vi "Signal CP Assigned Table.vi"(8 "CP Probability":dbl[][](array[numeric]), 9 "time":dbl[](array[numeric]), 10 "Change Point Array":T2, 11 "Assigned CP Profile plus":T1) -> (3 "CP Profile Table":string[][](table) caption="CP Table")   [LabVIEW 2018]
panel:
  out "サイズ 3":i32
  out "配列":string[][](array[string])
  out "要素":i32
  out "サイズ 2":i32
  out "サイズ":i32[](array[numeric])
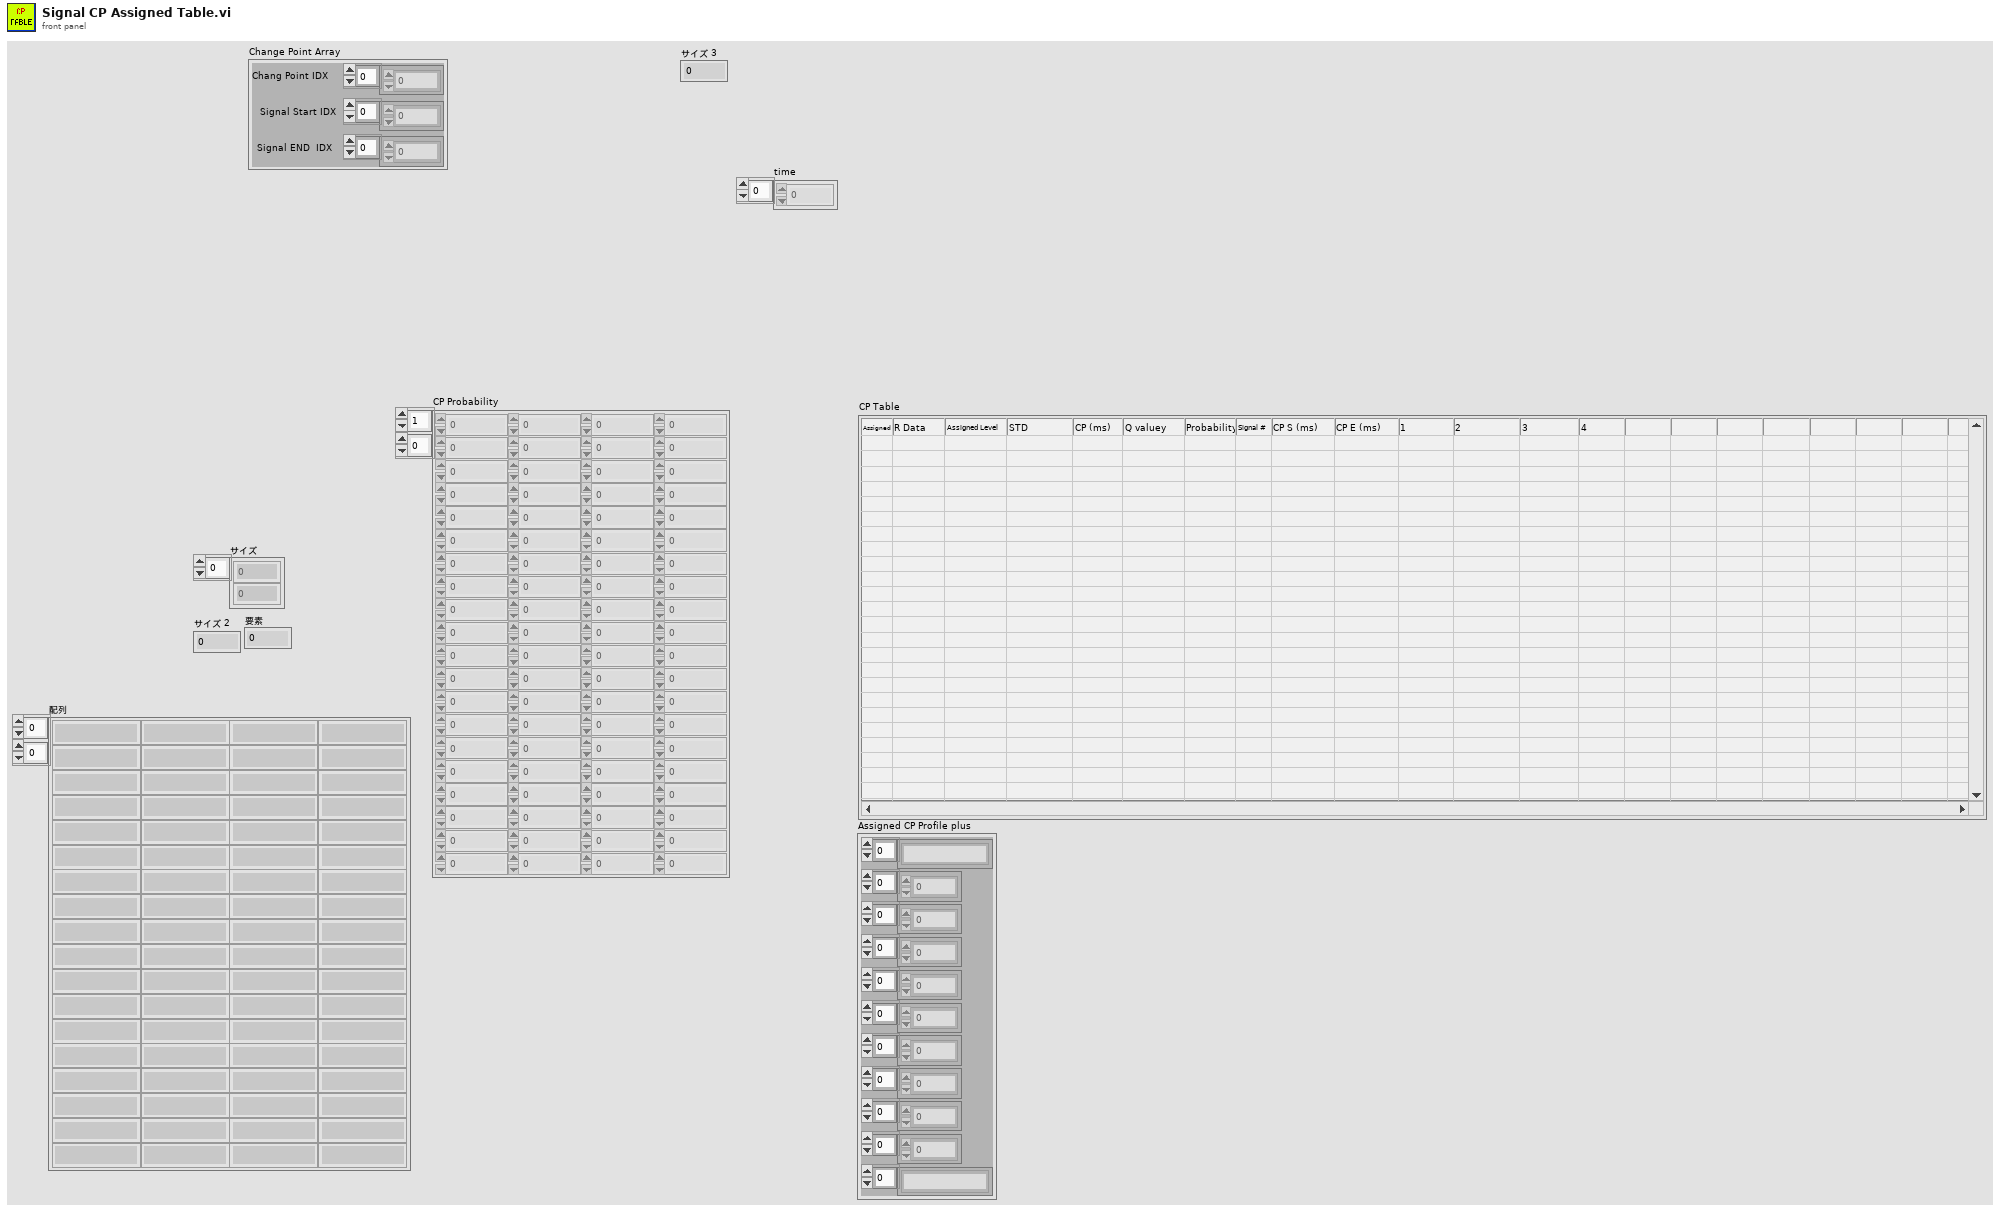
[diagram p1: front panel]
types:
  T1 = cluster{string[], dbl[], dbl[], dbl[], i32[], dbl[], dbl[], i32[], i32[], i32[], string[]}
  T2 = cluster{"Chang Point IDX":i32[], "Signal Start IDX":i32[], "Signal END  IDX":i32[]}
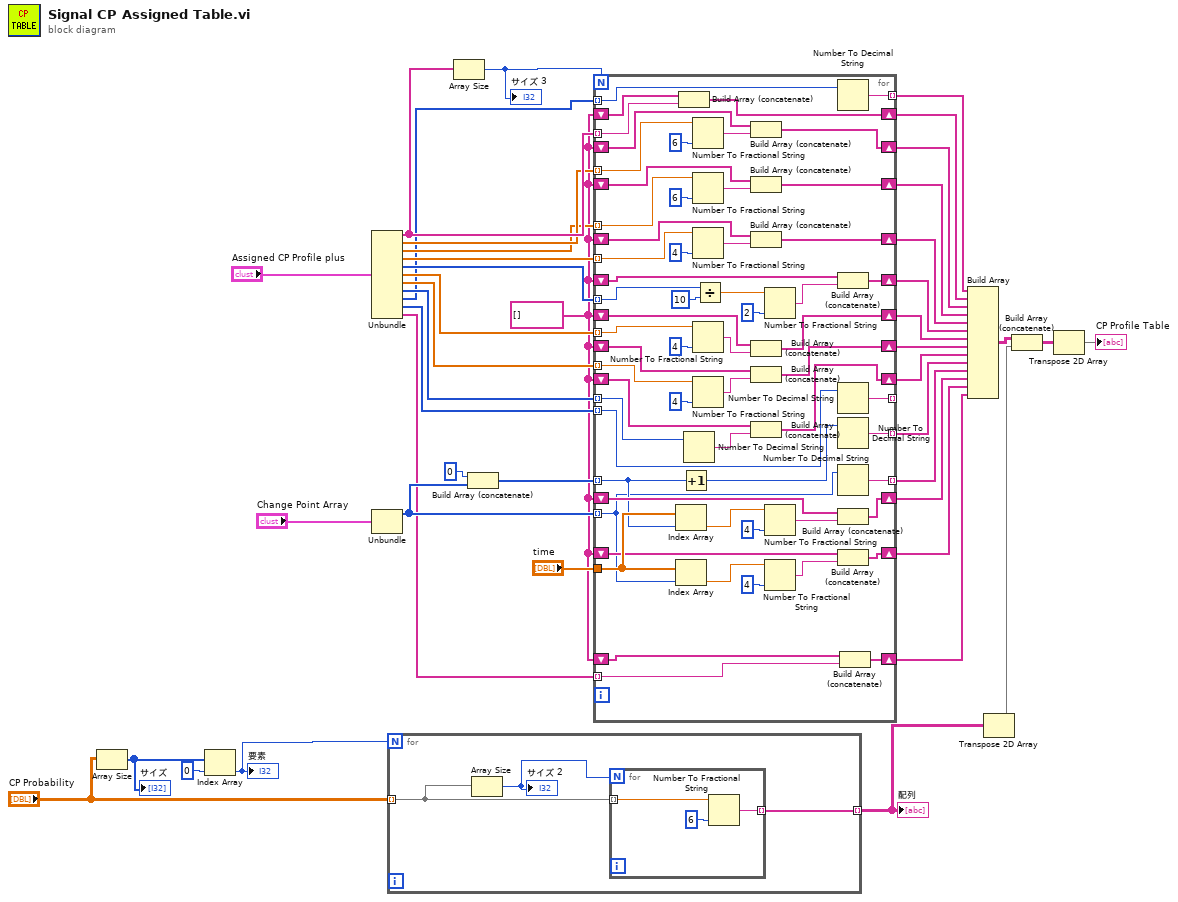
[diagram p0: block diagram]
diagram:
  w2 = string[] []
  n1 = Array Size(array="CP Probability") -> (size(s)=w33:i32[])
  "サイズ" <- w33
  n2 = Index Array(array=w33, index=0 ("指標")) -> (element=w31:i32)
  "要素" <- w31
  n3 = Unbundle("Assigned CP Profile plus") -> (w41:string[], w40:dbl[], w39:dbl[], w38:dbl[], w37:i32[], w36:dbl[], w35:dbl[], w34:i32[], w11:i32[], w10:i32[], w3:string[])
  n4 = Unbundle("Change Point Array") -> ("Chang Point IDX"=w28:i32[])  [unwired: 2 out]
  n5 = for {
    N: w31 -> [_]
    tunnel: "CP Probability" -> [w44] mode=indexing
    tunnel: [w43] -> w16 mode=indexing
    n6 = Array Size(array=w44) -> (size(s)=w45:i32)
    "サイズ 2" <- w45
    n7 = for {
      N: w45 -> [_]
      tunnel: w44 -> [w48] mode=indexing
      tunnel: [w47] -> w43 mode=indexing
      n8 = Number To Fractional String(number=w48, precision (6)=i16 6 ("精度（6）")) -> (F-format string=w47:string)  [unwired: 2 in]
    }
  }
  "配列" <- w16
  n9 = Array Size(array=w41) -> (size(s)=w42:i32)
  "サイズ 3" <- w42
  n10 = Build Array (concatenate)(0, w28) -> (w26:i32[])
  n11 = for {
    N: w42 -> [_]
    tunnel: w41 -> [w110] mode=indexing
    tunnel: w40 -> [w107] mode=indexing
    tunnel: w39 -> [w98] mode=indexing
    tunnel: w38 -> [w93] mode=indexing
    tunnel: w37 -> [w92] mode=indexing
    tunnel: w36 -> [w77] mode=indexing
    tunnel: w35 -> [w76] mode=indexing
    tunnel: w34 -> [w72] mode=indexing
    shift-right: [w109] -> w24
    shift-left: w2 -> [w108]
    shift-right: [w104] -> w23
    shift-left: w2 -> [w103]
    shift-right: [w100] -> w22
    shift-left: w2 -> [w99]
    shift-right: [w95] -> w21
    shift-left: w2 -> [w94]
    shift-right: [w87] -> w20
    shift-left: w2 -> [w86]
    shift-right: [w81] -> w19
    shift-left: w2 -> [w80]
    shift-right: [w79] -> w18
    shift-left: w2 -> [w78]
    shift-right: [w74] -> w5
    shift-left: w2 -> [w73]
    tunnel: w28 -> [w52] mode=indexing
    tunnel: w26 -> [w54] mode=indexing
    tunnel: "time" -> [w67]
    shift-right: [w68] -> w8
    shift-left: w2 -> [w63]
    shift-right: [w64] -> w9
    shift-left: w2 -> [w62]
    tunnel: w11 -> [w60] mode=indexing
    tunnel: [w59] -> w12 mode=indexing
    tunnel: w10 -> [w58] mode=indexing
    tunnel: [w57] -> _ mode=indexing
    tunnel: [w56] -> w6 mode=indexing
    tunnel: [w55] -> w7 mode=indexing
    tunnel: w3 -> [w51] mode=indexing
    shift-right: [w50] -> w1
    shift-left: w2 -> [w49]
    n12 = Index Array(array=w67, index=w54) -> (element=w69:dbl)
    n13 = Index Array(array=w67, index=w52) -> (element=w61:dbl)
    n14 = Build Array (concatenate)(w108, w110) -> (w109:string[])
    n15 = Increment(x=w54) -> (x+1=w53:i32)
    n16 = Number To Decimal String(number=w72) -> (decimal integer string=w75:string)  [unwired: 1 in]
    n17 = Number To Fractional String(number=w107, precision (6)=i16 6 ("精度（6）")) -> (F-format string=w105:string)  [unwired: 2 in]
    n18 = Number To Fractional String(number=w98, precision (6)=i16 6 ("精度（6）")) -> (F-format string=w101:string)  [unwired: 2 in]
    n19 = Number To Fractional String(number=w93, precision (6)=i16 4 ("精度（6）")) -> (F-format string=w96:string)  [unwired: 2 in]
    n20 = Number To Fractional String(number=w77, precision (6)=i16 4 ("精度（6）")) -> (F-format string=w84:string)  [unwired: 2 in]
    n21 = Number To Fractional String(number=w76, precision (6)=i16 4 ("精度（6）")) -> (F-format string=w82:string)  [unwired: 2 in]
    n22 = Divide(x=w92, y=10) -> (x/y=w89:dbl)
    n23 = Build Array (concatenate)(w103, w105) -> (w104:string[])
    n24 = Build Array (concatenate)(w99, w101) -> (w100:string[])
    n25 = Build Array (concatenate)(w94, w96) -> (w95:string[])
    n26 = Build Array (concatenate)(w80, w84) -> (w81:string[])
    n27 = Build Array (concatenate)(w78, w82) -> (w79:string[])
    n28 = Build Array (concatenate)(w73, w75) -> (w74:string[])
    n29 = Number To Fractional String(number=w89, precision (6)=i16 2 ("精度（6）")) -> (F-format string=w88:string)  [unwired: 2 in]
    n30 = Number To Fractional String(number=w69, precision (6)=i16 4 ("精度（6）")) -> (F-format string=w70:string)  [unwired: 2 in]
    n31 = Number To Fractional String(number=w61, precision (6)=i16 4 ("精度（6）")) -> (F-format string=w65:string)  [unwired: 2 in]
    n32 = Number To Decimal String(number=w60) -> (decimal integer string=w59:string)  [unwired: 1 in]
    n33 = Build Array (concatenate)(w86, w88) -> (w87:string[])
    n34 = Number To Decimal String(number=w58) -> (decimal integer string=w57:string)  [unwired: 1 in]
    n35 = Number To Decimal String(number=w53) -> (decimal integer string=w56:string)  [unwired: 1 in]
    n36 = Number To Decimal String(number=w52) -> (decimal integer string=w55:string)  [unwired: 1 in]
    n37 = Build Array (concatenate)(w63, w70) -> (w68:string[])
    n38 = Build Array (concatenate)(w62, w65) -> (w64:string[])
    n39 = Build Array (concatenate)(w49, w51) -> (w50:string[])
  }
  n40 = Build Array(w12, w24, w23, w22, w21, w20, w19, w18, w5, w6, w7, w8, w9, w1) -> (w15:string[][])
  n41 = Transpose 2D Array(2D array=w16) -> (transposed array=w13:string[][])
  n42 = Build Array (concatenate)(w15, w13) -> (w17:string[][])
  n43 = Transpose 2D Array(2D array=w17) -> (transposed array=→"CP Profile Table":string[][])
